vi "work2_cooker_module.vi"() -> ()   [LabVIEW 2026]
panel:
  out "Output":string
  in  "Cook Meal":bool
  in  "Burger":i16
  in  "Cook Burger":bool
  in  "Stop":bool
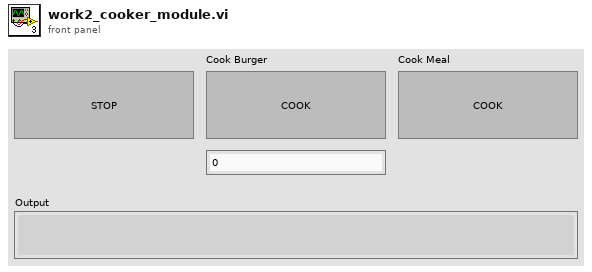
[diagram p1: front panel]
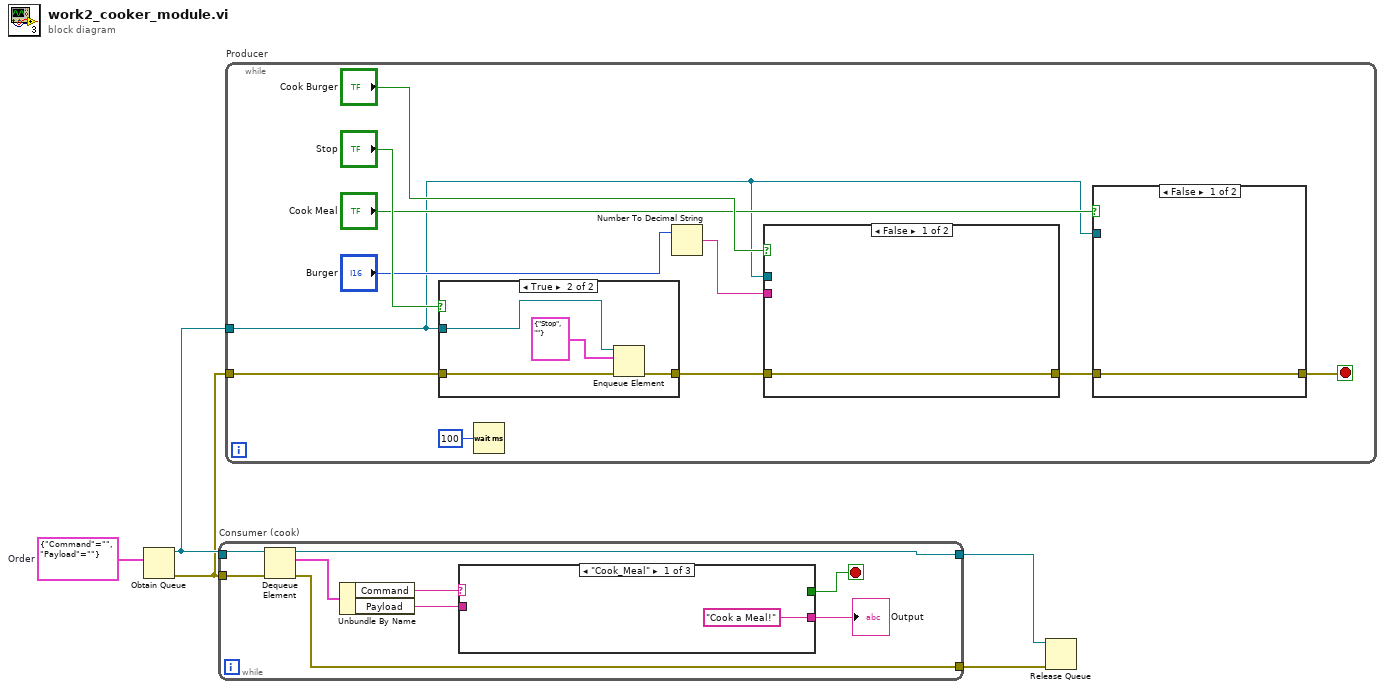
[diagram p0: block diagram]
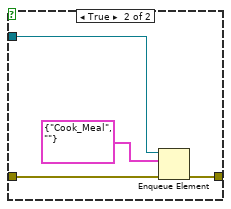
[diagram p2: hidden frame]
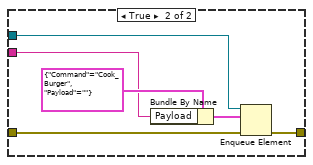
[diagram p3: hidden frame]
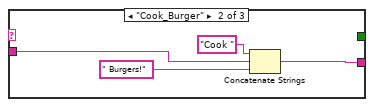
[diagram p5: hidden frame]
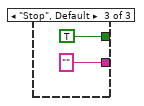
[diagram p6: hidden frame]
diagram:
  w3 = cluster{"Command":string, "Payload":string} {"Command"="", "Payload"=""}  # Order
  n1 = Obtain Queue(element data type=w3) -> (queue out=w2:refnum<queue>, error out=w1:errorcluster)  [unwired: 4 in, 1 out]
  n2 = while "Consumer (cook)" {
    tunnel: w2 -> [w14]
    tunnel: [w13] -> w5
    tunnel: w1 -> [w12]
    tunnel: [w11] -> w4
    stop <- w8 stop-if-true
    n3 = Dequeue Element(queue=w14, error in (no error)=w12) -> (queue out=w13:refnum<queue>, element=w10:cluster{"Command":string, "Payload":string}, error out=w11:errorcluster)  [unwired: 1 in, 1 out]
    n4 = Unbundle By Name(w10) -> ("Command"=w9:string, "Payload"=w6:string)
    n5 = case shown="\"Cook_Meal\"" w9 {
      tunnel: [_ _ TRUE] -> w8
      tunnel: ["Cook a Meal!" w16 ""] -> w7
      tunnel: w6 -> [_ w18 _]
      frame "Cook_Meal" {
      }
      frame "Cook_Burger" {
        n6 = Concatenate Strings("Cook " ("string"), w18, " Burgers!" ("string")) -> (w16:string)
      }
      frame "Stop", Default {
      }
    }
    "Output" <- w7
  }
  n7 = while "Producer" {
    tunnel: w2 -> [w24]
    tunnel: w1 -> [w22]
    stop <- w23 stop-if-true
    n8 = case shown="True" "Stop" {
      tunnel: w24 -> [_ w49]
      tunnel: [w45 w47] -> w30
      tunnel: w22 -> [w45 w46]
      frame False {
      }
      frame True {
        n9 = Enqueue Element(queue=w49, element=cluster{"Command":string, "Payload":string} {"Command"="Stop", "Payload"=""} ("Order"), error in (no error)=w46) -> (error out=w47:errorcluster)  [unwired: 1 in, 2 out]
      }
    }
    n10 = Wait (ms)(milliseconds to wait=u32 100) -> ()  [unwired: 1 out]
    n11 = Number To Decimal String(number="Burger") -> (decimal integer string=w27:string)  [unwired: 1 in]
    n12 = case shown="False" "Cook Burger" {
      tunnel: w24 -> [_ w44]
      tunnel: w30 -> [w38 w43]
      tunnel: w27 -> [_ w41]
      tunnel: [w38 w39] -> w25
      frame False {
      }
      frame True {
        n13 = Bundle By Name(cluster=cluster{"Command":string, "Payload":string} {"Command"="Cook_Burger", "Payload"=""} ("Order"), "Payload"=w41) -> (w40:cluster{"Command":string, "Payload":string})
        n14 = Enqueue Element(queue=w44, element=w40, error in (no error)=w43) -> (error out=w39:errorcluster)  [unwired: 1 in, 2 out]
      }
    }
    n15 = case shown="False" "Cook Meal" {
      tunnel: w24 -> [_ w37]
      tunnel: w25 -> [w33 w36]
      tunnel: [w33 w34] -> w23
      frame False {
      }
      frame True {
        n16 = Enqueue Element(queue=w37, element=cluster{"Command":string, "Payload":string} {"Command"="Cook_Meal", "Payload"=""} ("Order"), error in (no error)=w36) -> (error out=w34:errorcluster)  [unwired: 1 in, 2 out]
      }
    }
  }
  n17 = Release Queue(queue=w5, error in (no error)=w4) -> ()  [unwired: 1 in, 3 out]
